vi "Time.vi"(11 "字符串":string) -> (3 "连接的字符串":string)   [LabVIEW 2025]
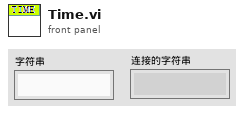
[diagram p1: front panel]
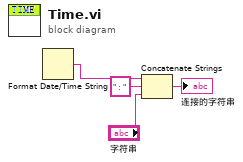
[diagram p0: block diagram]
diagram:
  n1 = Format Date/Time String() -> (date/time string=w4:string)  [unwired: 3 in]
  n2 = Concatenate Strings(w4, "：" ("字符串"), "字符串") -> (→"连接的字符串":string)
